vi "TEST - Periodic Trigger.vi"(8 "error in (no error)":errorcluster) -> (0 "error out":errorcluster, 2 "pass":bool)   [LabVIEW 2020]
uses:
  <vilib>/addons/_JKI Toolkits/Caraya/classes/Assert/Assert True.vi
  source/library/openg_time.lvlib
  <vilib>/addons/_JKI Toolkits/Caraya/classes/Test/Test.lvclass
  <vilib>/addons/_JKI Toolkits/Caraya/classes/Assert/Assert.lvclass
panel:
  out "sum":i16
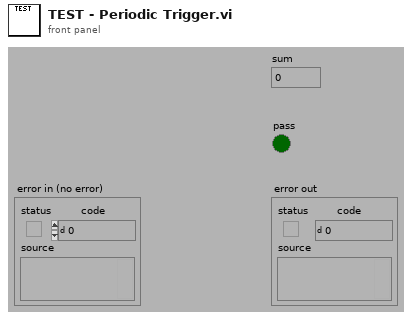
[diagram p1: front panel]
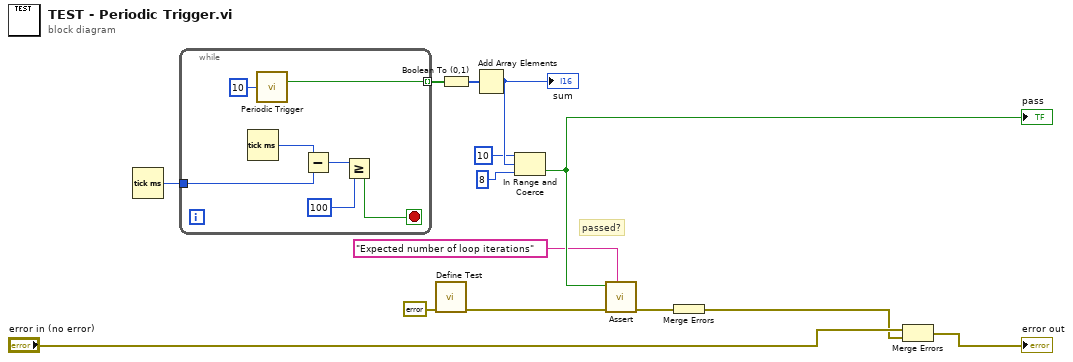
[diagram p0: block diagram]
diagram:
  # "passed?"
  n1 = Tick Count (ms)() -> (millisecond timer value=w11:u32)
  n2 = while {
    tunnel: w11 -> [w19]
    tunnel: [w20] -> w10 mode=indexing
    stop <- w16 stop-if-true
    n3 = Tick Count (ms)() -> (millisecond timer value=w15:u32)
    n4 = call "Periodic Trigger.vi"("time (ms)"=u32 10) -> ("Triggered"=w20:bool)  [unwired: 12 in, 2 out]
    n5 = Subtract(x=w15, y=w19) -> (x-y=w18:u32)
    n6 = Greater Or Equal?(x=w18, y=u32 100) -> (x >= y?=w16:bool)
  }
  n7 = call <vilib>:"Define Test.vi"("error in (no error)"=errorcluster {"status"=FALSE, "code"=0, "source"=""}) -> ("error out"=w3:errorcluster)  [unwired: 9 in, 1 out]
  n8 = Boolean To (0,1)(Boolean=w10) -> (0, 1=w9:i16[])
  n9 = Add Array Elements(numeric array=w9) -> (sum=w8:i16)
  "sum" <- w8
  n10 = In Range and Coerce(upper limit=i16 10 ("sum"), x=w8, lower limit=i16 8 ("sum")) -> (In Range?=w14:bool)  [unwired: 1 out]
  "pass" <- w14
  n11 = call-poly <vilib>:"Assert.vi"("Label"="Expected number of loop iterations" ("Label (VI Title)"), "error in (no error)"=w3, "True?"=w14) -> ("error out"=w4:errorcluster)  [unwired: 7 in, 1 out]
  n12 = Merge Errors(w4) -> (w1:errorcluster)
  n13 = Merge Errors("error in (no error)", w1) -> (→"error out":errorcluster)
